vi "Report App Info.vi"(8 "error in (no error)":errorcluster, 11 "Volatus Core in":refnum<class "Volatus Core.lvclass">) -> (0 "error out":errorcluster, 3 "Volatus Core out":refnum<class "Volatus Core.lvclass">)   [LabVIEW 2020, in "Volatus.lvlib" / "Volatus Core.lvclass"]
uses:
  Volatus Core.lvclass
  C:/dev/lv20CE/relink/lv-volatus/Volatus/Module/Module.lvclass
  Volatus Core.lvclass/Volatus Core.ctl
  Module/Module.lvclass/Module.ctl
  Module/Module.lvclass
  lv-vecto/Vecto/Node Config/Node Config.lvclass
  C:/dev/lv20CE/relink/lv-volatus/Volatus/Volatus Core/Volatus Core.lvclass
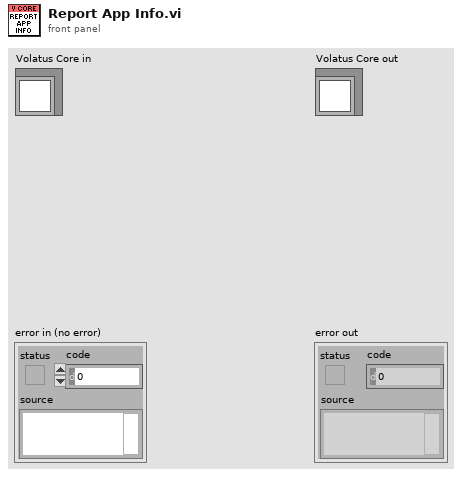
[diagram p1: front panel]
types:
  T1 = typedef "Volatus.lvlib/Volatus Core.lvclass/Config Type.ctl" = enum16{"App INI", "Memory", "Unconfigured"}
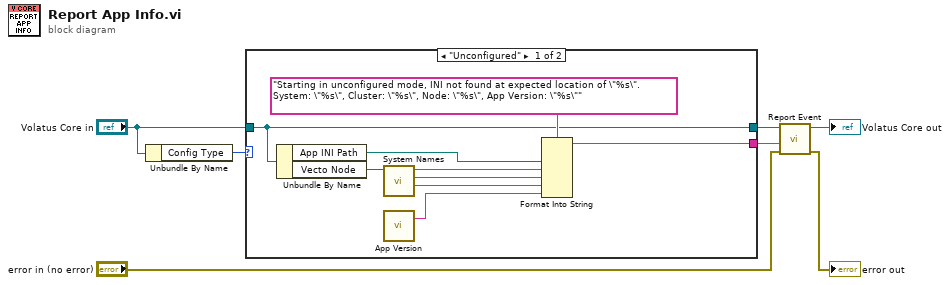
[diagram p0: block diagram]
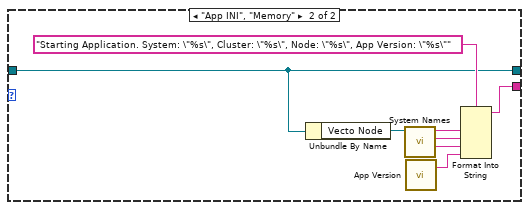
[diagram p2: hidden frame]
diagram:
  n1 = Unbundle By Name("Volatus Core in") -> ("Config Type"=w2:T1)
  n2 = case shown="\"Unconfigured\"" w2 {
    tunnel: [w9 w24] -> w4
    tunnel: "Volatus Core in" -> [w8 w17]
    tunnel: [w8 w17] -> w1
    frame "Unconfigured" {
      n3 = Unbundle By Name(w8) -> ("App INI Path"=w14:path, "Vecto Node"=w16:refnum<class "Node Config.lvclass">)
      n4 = call "System Names.vi"("Node Config in"=w16) -> ("Name"=w11:string, "Cluster"=w12:string, "System"=w13:string)  [unwired: 8 in]
      n5 = call "App Version.vi"() -> ("App Version"=w10:string)  [unwired: 3 in]
      n6 = Format Into String(format string="Starting in unconfigured mode, INI not found at expected location of \"%s\". System: \"%s\", Cluster: \"%s\", Node: \"%s\", App Version: \"%s\"", w14, w13, w12, w11, w10) -> (resulting string=w9:string)  [unwired: 2 in, 1 out]
    }
    frame "App INI", "Memory" {
      n7 = Unbundle By Name(w17) -> ("Vecto Node"=w21:refnum<class "Node Config.lvclass">)
      n8 = call "System Names.vi"("Node Config in"=w21) -> ("Name"=w18:string, "Cluster"=w19:string, "System"=w20:string)  [unwired: 8 in]
      n9 = call "App Version.vi"() -> ("App Version"=w23:string)  [unwired: 3 in]
      n10 = Format Into String(format string="Starting Application. System: \"%s\", Cluster: \"%s\", Node: \"%s\", App Version: \"%s\"", w20, w19, w18, w23) -> (resulting string=w24:string)  [unwired: 2 in, 1 out]
    }
  }
  n11 = call "Report Event.vi"("error in (no error)"="error in (no error)", "Message"=w4, "Module in"=w1) -> ("error out"=→"error out":errorcluster, "Module out"=→"Volatus Core out":refnum<class "Volatus Core.lvclass">)  [unwired: 7 in]
